vi "Write Graph-Chart Axis Labels.vi"(8 "error in":errorcluster, 9 "Y Axis":string, 10 "X Axis":string, 11 "Graph / Chart Reference in":refnum<vi>) -> (0 "error out":errorcluster, 3 "Graph / Chart Reference out":refnum<vi>)   [LabVIEW 2020, in "G-Unicode.lvlib"]
uses:
  G-Unicode.lvlib
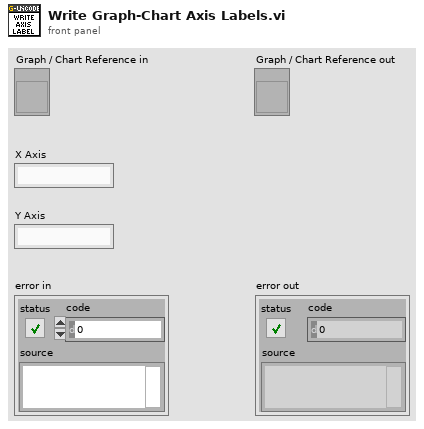
[diagram p1: front panel]
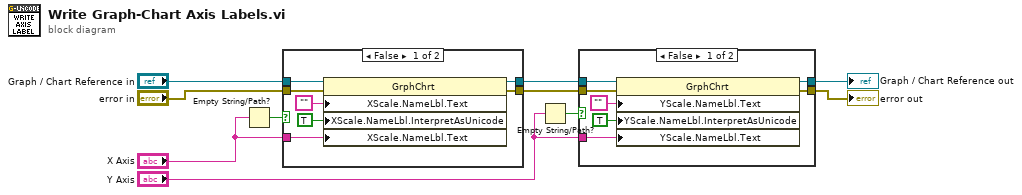
[diagram p0: block diagram]
diagram:
  n1 = Empty String/Path?(string/path="X Axis") -> (empty?=w4:bool)
  n2 = case shown="False" w4 {
    tunnel: "Graph / Chart Reference in" -> [w15 w19]
    tunnel: "error in" -> [w14 w18]
    tunnel: "X Axis" -> [w13 _]
    tunnel: [w12 w19] -> w8
    tunnel: [w11 w18] -> w6
    frame False {
      n3 = property class="GrphChrt"(reference=w15, error in=w14, "XScale.NameLbl.Text"="" ("Value"), "XScale.NameLbl.InterpretAsUnicode"=TRUE ("Text.Interpret As Unicode"), "XScale.NameLbl.Text"=w13) -> (reference out=w12:refnum<vi>, error out=w11:errorcluster)
    }
    frame True {
    }
  }
  n4 = Empty String/Path?(string/path="Y Axis") -> (empty?=w3:bool)
  n5 = case shown="False" w3 {
    tunnel: w8 -> [w26 w28]
    tunnel: [w25 w28] -> w7
    tunnel: w6 -> [w24 w27]
    tunnel: [w23 w27] -> w5
    tunnel: "Y Axis" -> [w22 _]
    frame False {
      n6 = property class="GrphChrt"(reference=w26, error in=w24, "YScale.NameLbl.Text"="" ("Value"), "YScale.NameLbl.InterpretAsUnicode"=TRUE ("Y Scale.Name Label.Interpret As Unicode"), "YScale.NameLbl.Text"=w22) -> (reference out=w25:refnum<vi>, error out=w23:errorcluster)
    }
    frame True {
    }
  }
  "error out" <- w5
  "Graph / Chart Reference out" <- w7
